vi "CreateReferences.vi"(7 "Coorinate System?":bool, 8 "error in (no error)":errorcluster, 9 "AxisArray_FromConf":string[](array[string]), 10 "Axis Name":string="Axis 1", 11 "SoftmotionAxis in":refnum<class "SoftmotionAxis.lvclass">) -> (0 "error out":errorcluster, 3 "SoftmotionAxis out":refnum<class "SoftmotionAxis.lvclass">)   [LabVIEW 2017, in "SoftmotionAxis.lvclass"]
uses:
  SoftmotionAxis.lvclass
  <vilib>/Motion/PropertyNodes/nimc.createStraightLineMoveInstance.axis.vi
  <vilib>/Motion/PropertyNodes/nimc.createReferenceMoveInstance.axis.vi
  <vilib>/Motion/PropertyNodes/nimc.createStopMoveInstance.axis.vi
  <vilib>/Motion/PropertyNodes/nimc.destroyInterfaceInstance.vi
  <vilib>/Motion/PropertyNodes/nimc.createStraightLineMoveInstance.coordinate.vi
  <vilib>/Motion/PropertyNodes/nimc.createStopMoveInstance.coordinate.vi
  <resource>/objmgr/nimcai.rc
  <resource>/objmgr/nimotion.rc
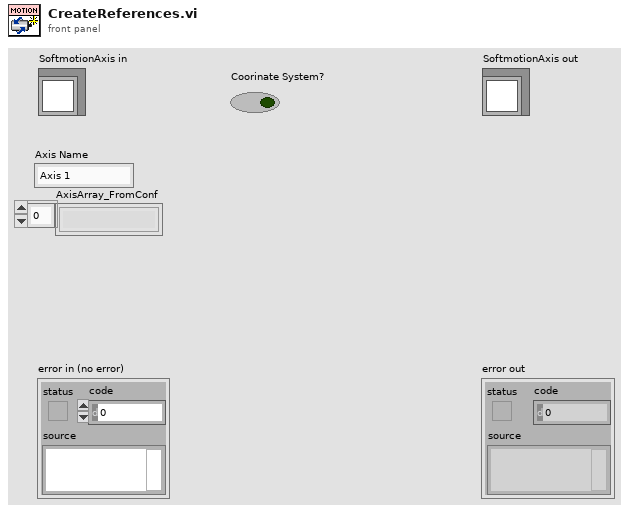
[diagram p1: front panel]
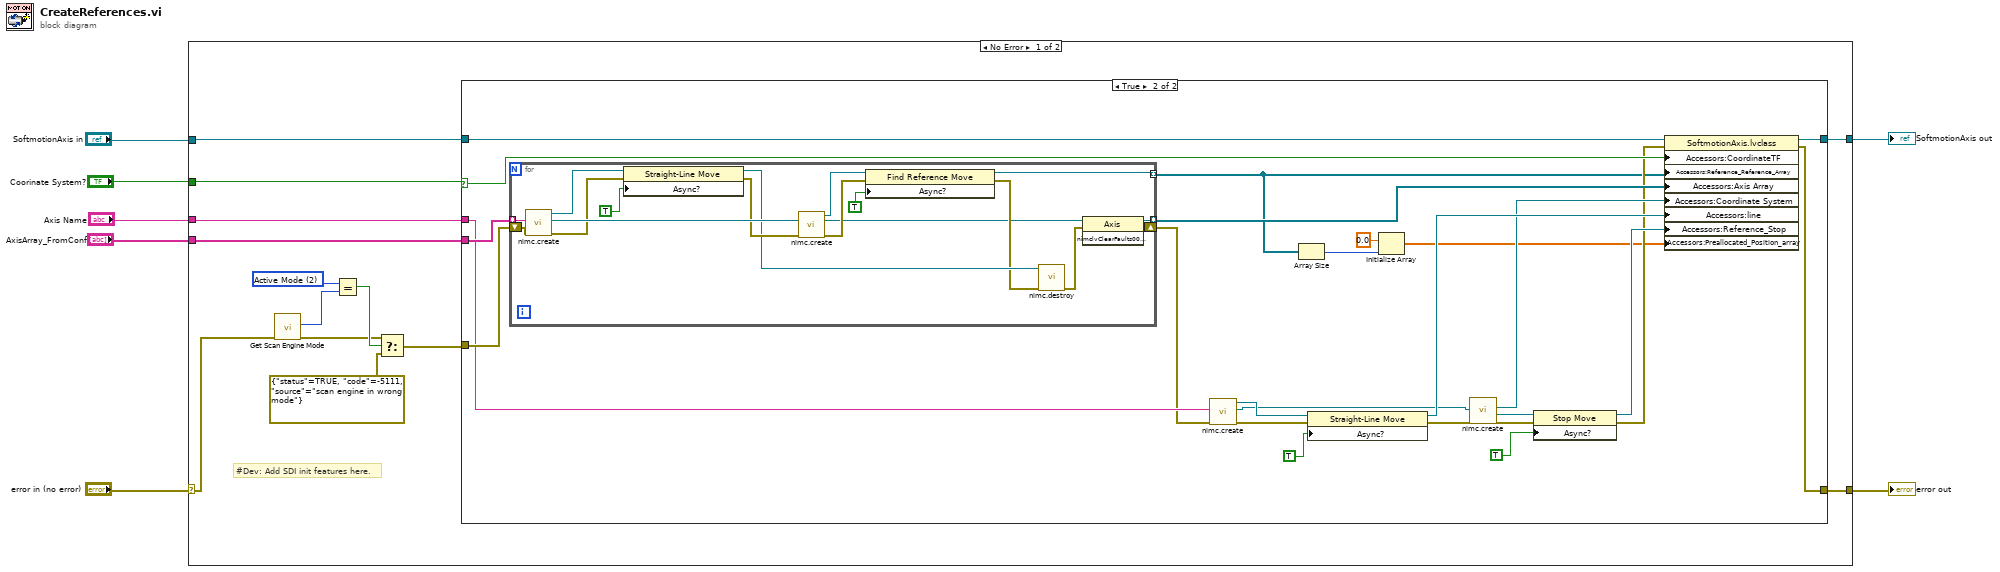
[diagram p0: block diagram]
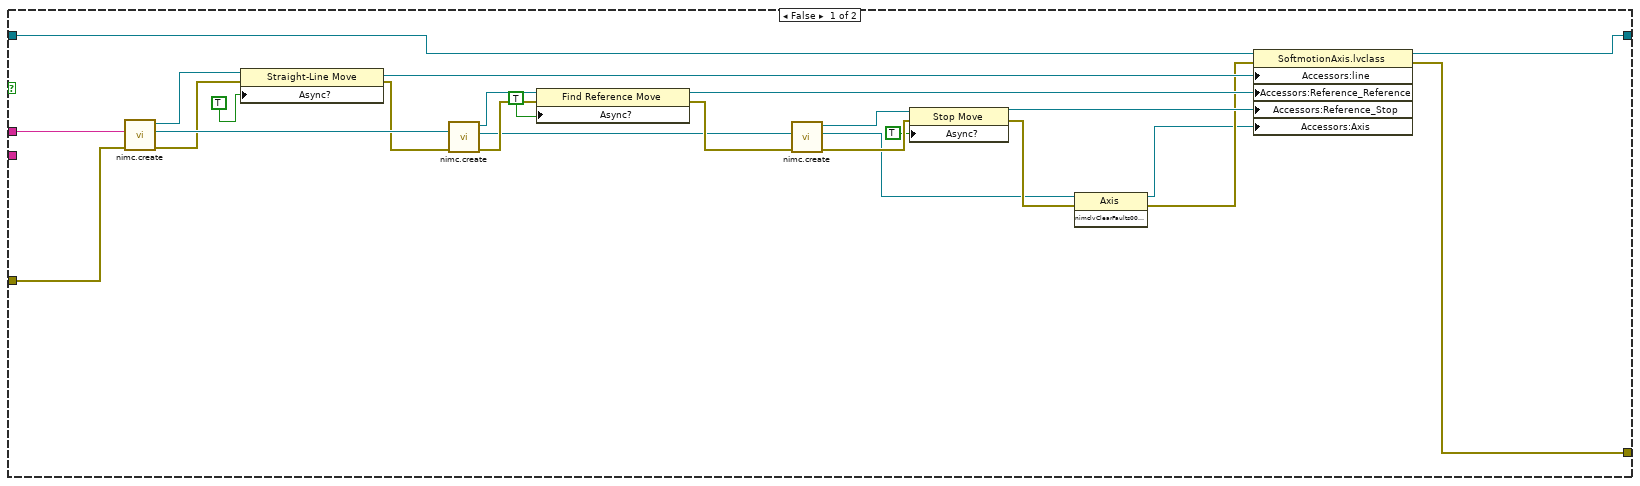
[diagram p2: hidden frame]
diagram:
  n1 = case shown="No Error" "error in (no error)" {
    selector: "error in (no error)" -> [w18 w89]
    tunnel: [w17 w89] -> w6
    tunnel: [w19 w88] -> w4
    tunnel: "SoftmotionAxis in" -> [w15 w88]
    tunnel: "Axis Name" -> [w16 _]
    tunnel: "Coorinate System?" -> [w9 _]
    tunnel: "AxisArray_FromConf" -> [w8 _]
    frame No Error {
      w13 = 2 items=["Configuration Mode"=1, "Active Mode"=2] ("mode (Active Mode)")
      # "#Dev: Add SDI init features here."
      n2 = call <vilib>:"Get Scan Engine Mode.vi"("error in (no error)"=w18) -> ("error out"=w11:errorcluster, "mode"=w14:i32)  [unwired: 9 in]
      n3 = Equal?(x=w13, y=w14) -> (x = y?=w12:bool)
      n4 = Select(t=w11, s=w12, f=errorcluster {"status"=TRUE, "code"=-5111, "source"="scan engine in wrong mode"} ("error in (no error)")) -> (s? t:f=w20:errorcluster)
      n5 = case shown="True" w9 {
        selector: w9 -> [_ w60]
        tunnel: w20 -> [w45 w70]
        tunnel: [w44 w69] -> w19
        tunnel: [w24 w55] -> w17
        tunnel: w16 -> [w42 w63]
        tunnel: w15 -> [w39 w68]
        tunnel: w8 -> [_ w67]
        frame False {
          n6 = call-poly <vilib>:"nimc.create.vi"("error in"=w45, "axis"=w42) -> ("error out"=w33:errorcluster, "axis out"=w41:refnum<k21>, "line"=w34:refnum<k20>)  [unwired: 7 in]
          n7 = property class="Straight-Line Move"(reference=w34, error in=w33, "Async?"=TRUE) -> (reference out=w43:refnum<k20>, error out=w40:errorcluster)
          n8 = call-poly <vilib>:"nimc.create.vi"("error in"=w40, "axis"=w41) -> ("error out"=w37:errorcluster, "axis out"=w30:refnum<k21>, "reference"=w38:refnum<k20>)  [unwired: 7 in]
          n9 = property class="Find Reference Move"(reference=w38, error in=w37, "Async?"=TRUE) -> (reference out=w36:refnum<k20>, error out=w31:errorcluster)
          n10 = call-poly <vilib>:"nimc.create.vi"("error in"=w31, "axis"=w30) -> ("error out"=w27:errorcluster, "axis out"=w22:refnum<k21>, "stop"=w28:refnum<k20>)  [unwired: 7 in]
          n11 = property class="Stop Move"(reference=w28, error in=w27, "Async?"=TRUE) -> (reference out=w29:refnum<k20>, error out=w23:errorcluster)
          n12 = invoke class="Axis" method="nimclvClearFaults00A10001"(reference=w22, error in=w23) -> (reference out=w21:refnum<k21>, error out=w25:errorcluster)  [unwired: 1 in, 1 out]
          n13 = property class="SoftmotionAxis.lvclass"(reference=w39, error in=w25, "Accessors:line"=w43, "Accessors:Reference_Reference"=w36, "Accessors:Reference_Stop"=w29, "Accessors:Axis"=w21) -> (reference out=w44:refnum<class "SoftmotionAxis.lvclass">, error out=w24:errorcluster)
        }
        frame True {
          n14 = for {
            shift-right: [w86] -> w62
            shift-left: w70 -> [w87]
            tunnel: w67 -> [w77] mode=indexing
            tunnel: [w76] -> w49 mode=indexing
            tunnel: [w75] -> w59 mode=indexing
            n15 = call-poly <vilib>:"nimc.create.vi"("error in"=w87, "axis"=w77) -> ("error out"=w79:errorcluster, "axis out"=w85:refnum<k21>, "line"=w80:refnum<k20>)  [unwired: 7 in]
            n16 = property class="Straight-Line Move"(reference=w80, error in=w79, "Async?"=TRUE) -> (reference out=w74:refnum<k20>, error out=w84:errorcluster)
            n17 = call-poly <vilib>:"nimc.create.vi"("error in"=w84, "axis"=w85) -> ("error out"=w82:errorcluster, "axis out"=w71:refnum<k21>, "reference"=w83:refnum<k20>)  [unwired: 7 in]
            n18 = property class="Find Reference Move"(reference=w83, error in=w82, "Async?"=TRUE) -> (reference out=w76:refnum<k20>, error out=w73:errorcluster)
            n19 = call-poly <vilib>:"nimc.destroy.vi"("error in"=w73, "motion handle"=w74) -> ("error out"=w72:errorcluster)  [unwired: 9 in]
            n20 = invoke class="Axis" method="nimclvClearFaults00A10001"(reference=w71, error in=w72) -> (reference out=w75:refnum<k21>, error out=w86:errorcluster)  [unwired: 1 in, 1 out]
          }
          n21 = call-poly <vilib>:"nimc.create.vi"("error in"=w62, "coordinate"=w63) -> ("error out"=w65:errorcluster, "coordinate out"=w58:refnum<k21>, "line"=w64:refnum<k20>)  [unwired: 7 in]
          n22 = Array Size(array=w49) -> (size(s)=w48:i32)
          n23 = property class="Straight-Line Move"(reference=w64, error in=w65, "Async?"=TRUE) -> (reference out=w61:refnum<k20>, error out=w56:errorcluster)
          n24 = Initialize Array(0.0 ("element"), w48) -> (w47:dbl[])
          n25 = call-poly <vilib>:"nimc.create.vi"("error in"=w56, "coordinate"=w58) -> ("error out"=w51:errorcluster, "coordinate out"=w57:refnum<k21>, "stop"=w53:refnum<k20>)  [unwired: 7 in]
          n26 = property class="Stop Move"(reference=w53, error in=w51, "Async?"=TRUE) -> (reference out=w52:refnum<k20>, error out=w50:errorcluster)
          n27 = property class="SoftmotionAxis.lvclass"(reference=w68, error in=w50, "Accessors:CoordinateTF"=w60, "Accessors:Reference_Reference_Array"=w49, "Accessors:Axis Array"=w59, "Accessors:Coordinate System"=w57, "Accessors:line"=w61, "Accessors:Reference_Stop"=w52, "Accessors:Preallocated_Position_array"=w47) -> (reference out=w69:refnum<class "SoftmotionAxis.lvclass">, error out=w55:errorcluster)
        }
      }
    }
    frame Error {
    }
  }
  "error out" <- w6
  "SoftmotionAxis out" <- w4
